vi "KeybdEventSerializerLUT.vi"(6 "SampleData":T4={"axis info"={"Horizontal"=0, "Vertical"=0, "Scrolling"=0}, "button info"={"button 1"=FALSE, "button 2"=FALSE, "button 3"=FALSE, "button 4"=FALSE}, "Relative Time (User Event)"=0.0, "Sample Number"=0, "Relative Time (Frame 0)"=0.0, "key mode"=enum."ABSOLUTE", "Frame Number"=0, "Keyboard KeysPressed"=[], "Keyboard No Op"=FALSE}, 8 "error in (no error)":errorcluster, 9 "Iteration":u32, 10 "keyType":T2=enum."RIGHT", 11 "VirtualKeyLUTSelector":T1) -> (0 "error out":errorcluster, 1 "Samples":i32, 2 "Unimplemented":bool, 3 "cluster":T3)   [LabVIEW 2026, in "dependencies.lvlib"]
uses:
  dependencies.lvlib
  KeyType.ctl
  KeyboardAndMouseDataAcquisition.ctl
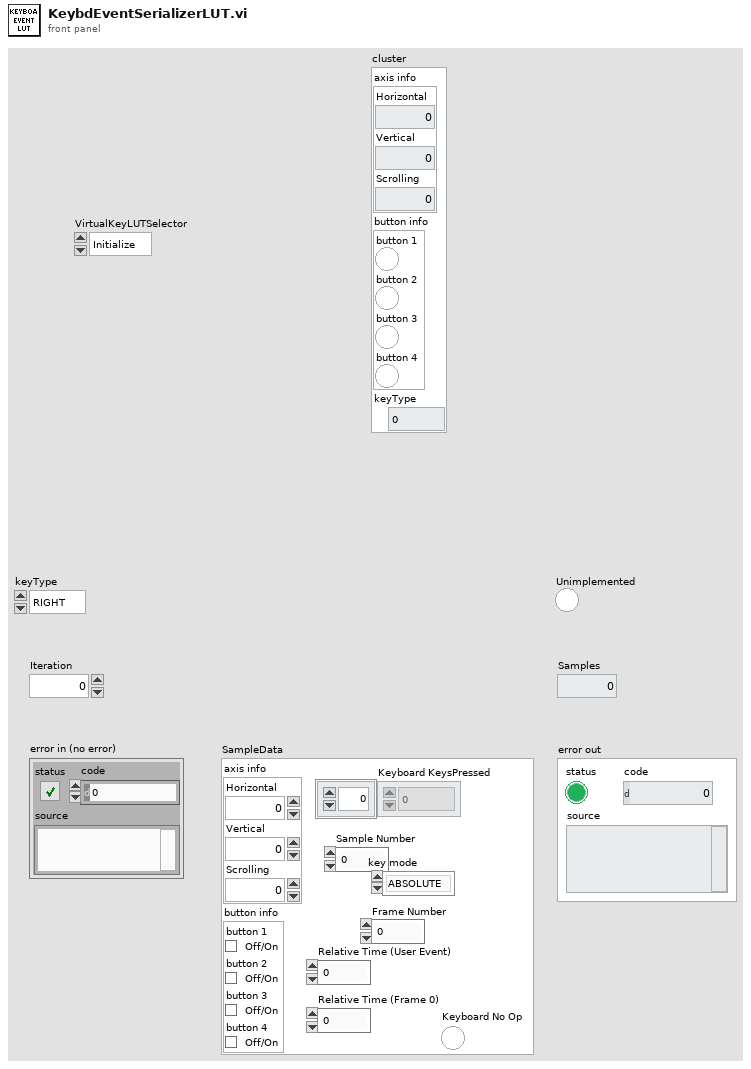
[diagram p1: front panel]
types:
  T1 = typedef "dependencies.lvlibp/LUTVirtualKeySelector.ctl" = enum16{"Initialize", "Get Keyboard Event", "Set Keyboard Event"}
  T2 = typedef "dependencies.lvlib/KeyType.ctl" = enum16{"0", "1", "2", "3", "4", "5", "6", "7", "8", "9", "A", "B", "C", "D", "E", "F", "G", "H", "I", "J", "K", "L", "M", "N", "O", "P", "Q", "R", "S", "T", "U", "V", "W", "X", "Y", "Z", "F1", "F2", "F3", "F4", "F5", "F6", "F7", "F8", "F9", "F10", "F11", "F12", "F13", "F14", "F15", "ADD", "BACK", "BACKSLASH", "CAPITAL", "COMMA", "DECIMAL", "DELETE", "DIVIDE", "DOWN", "END", "EQUALS", "ESCAPE", "GRAVE (`)", "HOME", "INSERT", "LBRACKET", "LCONTROL", "LEFT", "L ALT", "LSHIFT", "LWIN", "MINUS", "MULTIPLY", "NEXT", "NUMLOCK", "NUMPAD_0", "NUMPAD_1", "NUMPAD_2", "NUMPAD_3", "NUMPAD_4", "NUMPAD_5", "NUMPAD_6", "NUMPAD_7", "NUMPAD_8", "NUMPAD_9", "PAUSE", "PERIOD", "PRIOR (PG UP)", "RBRACKET", "RCONTROL", "RETURN", "RIGHT", "R ALT", "RSHIFT", "RWIN", "SCROLL", "SEMICOLON", "SLASH", "SPACE", "SUBTRACT", "TAB", "UP", "ENTER (num pad)", "' (quote)"}
  T3 = cluster{"axis info":cluster{"Horizontal":i32, "Vertical":i32, "Scrolling":i32}, "button info":cluster{"button 1":bool, "button 2":bool, "button 3":bool, "button 4":bool}, "keyType":T2}
  T4 = typedef "dependencies.lvlib/KeyboardAndMouseDataAcquisition.ctl" = cluster{"axis info":cluster{"Horizontal":i32, "Vertical":i32, "Scrolling":i32}, "button info":cluster{"button 1":bool, "button 2":bool, "button 3":bool, "button 4":bool}, "Relative Time (User Event)":dbl, "Sample Number":u32, "Relative Time (Frame 0)":dbl, "key mode":enum16{"RELATIVE", "ABSOLUTE"}, "Frame Number":u32, "Keyboard KeysPressed":T2[], "Keyboard No Op":bool}
  T5 = cluster{"Horizontal":i32, "Vertical":i32, "Scrolling":i32}
  T6 = cluster{"button 1":bool, "button 2":bool, "button 3":bool, "button 4":bool}
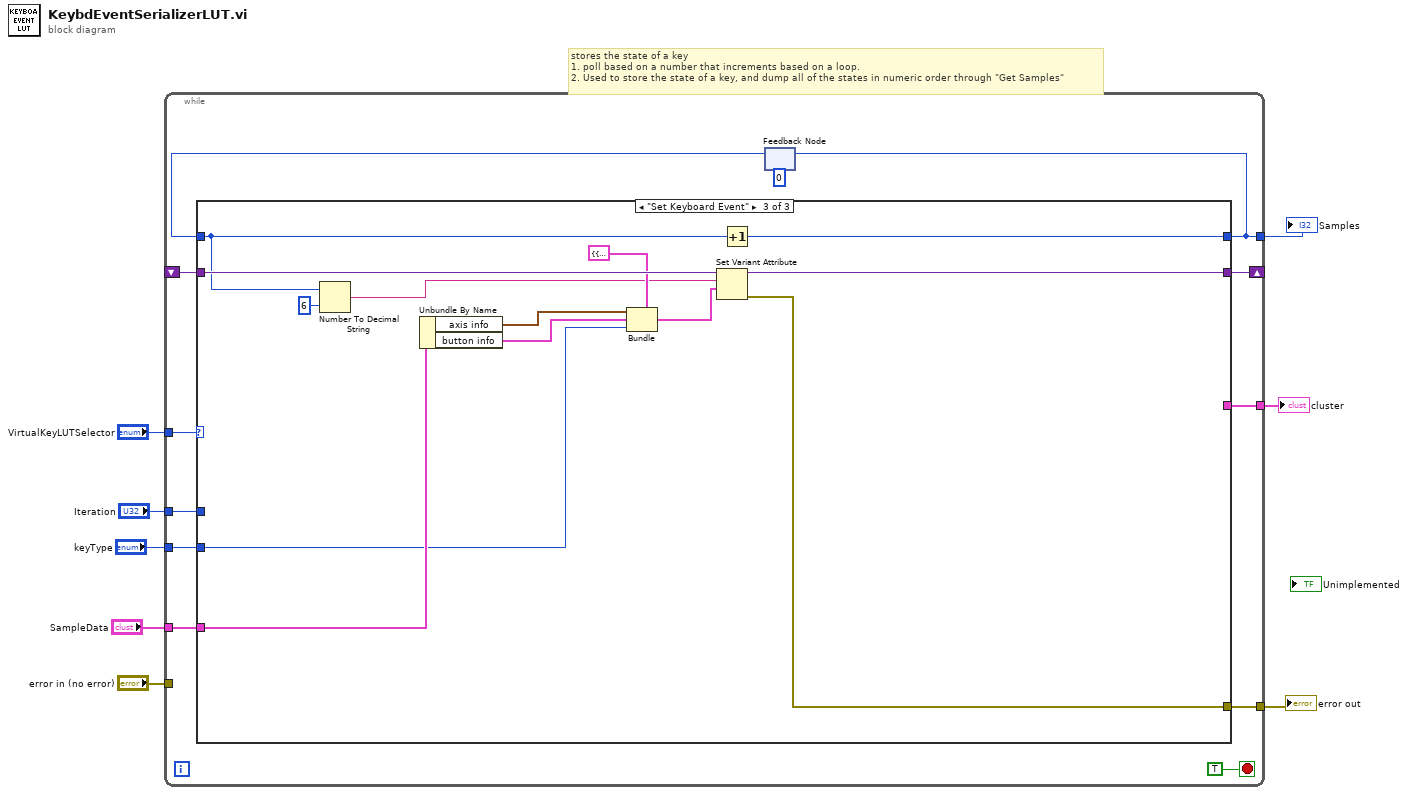
[diagram p0: block diagram]
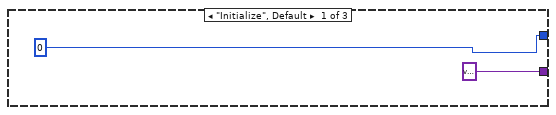
[diagram p2: hidden frame]
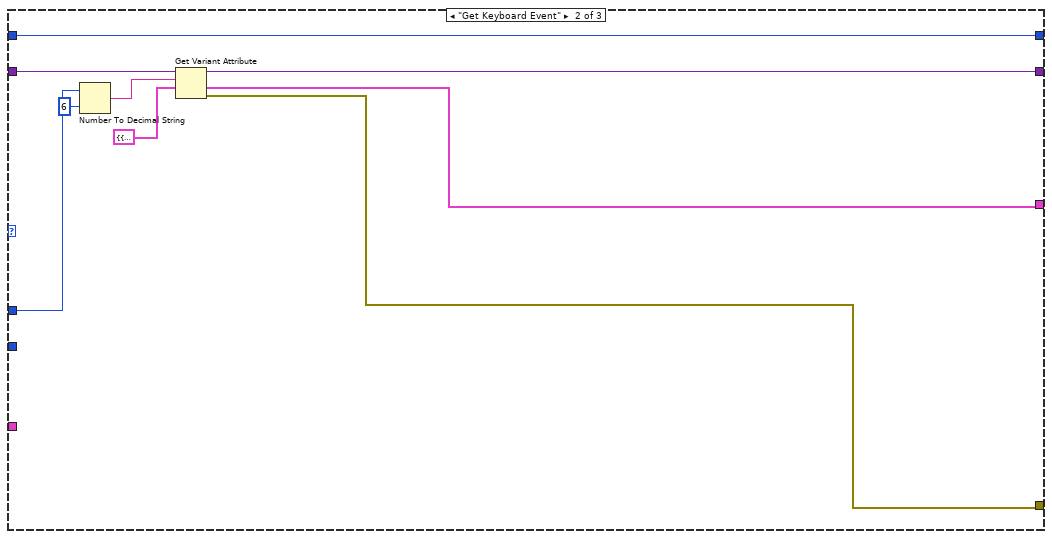
[diagram p3: hidden frame]
diagram:
  # "stores the state of a key\n1. poll based on a number that increments based on a loop.\n2. Used to store the state of a key, and dump all of the states in numeric order through \"Get Samples\""
  n1 = while {
    tunnel: "VirtualKeyLUTSelector" -> [w19]
    shift-right: [w18] -> _
    shift-left: _ -> [w17]
    tunnel: "Iteration" -> [w16]
    tunnel: [w15] -> w8
    tunnel: "keyType" -> [w14]
    tunnel: [w13] -> w2
    tunnel: "error in (no error)" -> [_]
    tunnel: [w10] -> w4
    tunnel: "SampleData" -> [w9]
    stop <- TRUE stop-if-true
    n2 = feedback #1(0 ("Index")) -> (w11:i32)
    n3 = case shown="\"Set Keyboard Event\"" w19 {
      tunnel: [variant w29 w43] -> w18
      tunnel: w17 -> [_ w31 w44]
      tunnel: w16 -> [_ w25 _]
      tunnel: [_ w28 w41] -> w15
      tunnel: w14 -> [_ _ w35]
      tunnel: [_ w27 _] -> w13
      tunnel: [0 ("Index") w30 w42] -> w10
      tunnel: w11 -> [_ w30 w33]
      tunnel: w9 -> [_ _ w40]
      frame "Initialize", Default {
      }
      frame "Get Keyboard Event" {
        n4 = Number To Decimal String(number=w25, width (-)=i16 6) -> (decimal integer string=w24:string)
        n5 = Get Variant Attribute(Variant=w31, name=w24, default value (empty Variant)=T3 {"axis info"={"Horizontal"=0, "Vertical"=0, "Scrolling"=0}, "button info"={"button 1"=FALSE, "button 2"=FALSE, "button 3"=FALSE, "button 4"=FALSE}, "keyType"=enum."RIGHT"} ("cluster")) -> (duplicate Variant=w29:variant, value=w27:T3, error out=w28:errorcluster)  [unwired: 1 in, 1 out]
      }
      frame "Set Keyboard Event" {
        n6 = Number To Decimal String(number=w33, width (-)=i16 6) -> (decimal integer string=w32:string)
        n7 = Unbundle By Name(w40) -> ("axis info"=w37:T5, "button info"=w36:T6)
        n8 = Bundle(cluster=T3 {"axis info"={"Horizontal"=0, "Vertical"=0, "Scrolling"=0}, "button info"={"button 1"=FALSE, "button 2"=FALSE, "button 3"=FALSE, "button 4"=FALSE}, "keyType"=enum."RIGHT"}, "axis info"=w37, "button info"=w36, "keyType"=w35) -> (w39:T3)
        n9 = Set Variant Attribute(Variant=w44, name=w32, value=w39) -> (Variant out=w43:variant, error out=w41:errorcluster)  [unwired: 1 in, 1 out]
        n10 = Increment(x=w33) -> (x+1=w42:i32)
      }
    }
    n11 = feedback-in #1(w10) -> ()
  }
  "error out" <- w8
  "Samples" <- w4
  "cluster" <- w2
